vi "Open Library References.vi"(8 "error in":errorcluster, 11 "Project Manager in":refnum<class "Project Manager.lvclass">) -> (0 "error out":errorcluster, 3 "Project Manager out":refnum<class "Project Manager.lvclass">)   [LabVIEW 2026, in "Project Manager.lvclass"]
doc: "Open references to lvlib elements in the project."
uses:
  Project Manager.lvclass
  Project Manager.lvclass/Project Manager.ctl
  Interfaces/ILogger/ILogger Messages/Log Msg/Log Msg.lvclass/Log Msg.ctl
  <vilib>/ActorFramework/Message Enqueuer/Message Enqueuer.lvclass/Message Enqueuer.ctl
  <vilib>/ActorFramework/Message Enqueuer/Enqueue.vi
  Interfaces/ILogger/ILogger Messages/Log Msg/Log Msg.lvclass
  <vilib>/ActorFramework/Message Priority Queue/Priority Enqueue.vi
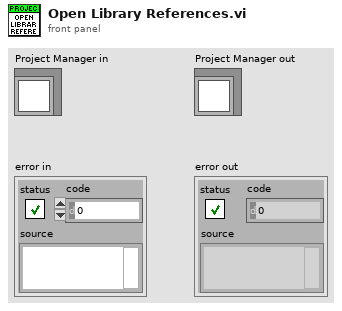
[diagram p1: front panel]
types:
  T1 = typedef "Log Entry--cluster.ctl" = cluster{"Time":timestamp, "Message":string}
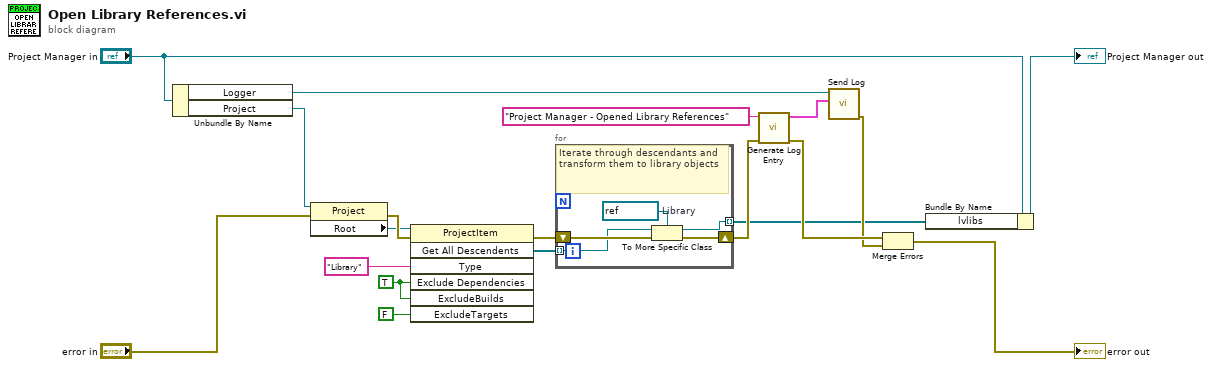
[diagram p0: block diagram]
diagram:
  w11 = TRUE ("ExcludeDependencies")
  n1 = Unbundle By Name("Project Manager in") -> ("Logger"=w3:refnum<class "Message Enqueuer.lvclass">, "Project"=w4:refnum<vi>)
  n2 = property class="Project"(reference=w4, error in="error in") -> (error out=w19:errorcluster, "Root"=w12:refnum<vi>)  [unwired: 1 out]
  n3 = invoke class="ProjectItem" method="Get All Descendents"(reference=w12, error in=w19, "Type"="Library", "Exclude Dependencies"=w11, "ExcludeBuilds"=w11, "ExcludeTargets"=FALSE) -> (error out=w18:errorcluster, "All Descendents"=w8:refnum<vi>[])  [unwired: 1 in, 5 out]
  n4 = for {
    tunnel: w8 -> [w21] mode=indexing
    shift-right: [w23] -> w16
    shift-left: w18 -> [w24]
    tunnel: [w20] -> w6 mode=indexing
    w22 = refnum<vi> refnum  # Library
    # "Iterate through descendants and transform them to library objects"
    n5 = To More Specific Class(target class=w22, reference=w21, error in=w24) -> (specific class reference=w20:refnum<vi>, error out=w23:errorcluster)
  }
  n6 = call "Generate Log Entry.vi"("error in"=w16, "Message"="Project Manager - Opened Library References") -> ("error out"=w15:errorcluster, "Log Entry"=w2:T1)  [unwired: 8 in]
  n7 = call "Send Log.vi"("Log Entry"=w2, "Message Enqueuer"=w3) -> ("error out"=w13:errorcluster)  [unwired: 8 in, 1 out]
  n8 = Merge Errors(w15, w13) -> (→"error out":errorcluster)
  n9 = Bundle By Name(cluster="Project Manager in", "lvlibs"=w6) -> (→"Project Manager out":refnum<class "Project Manager.lvclass">)
